vi "DiffDriveTrainSim_Update.vi"(6 "dT_Seconds":dbl=0.02, 11 "in DiffDriveTrainSim":T1 {"m_Motor"."Jr_KgM2" format="%13.5p"; "m_Motor"."L_H" format="%13.5p"; "m_Motor"."Kt_NMPerAmp" format="%13.5p"; "m_Motor"."KvINV_RadPerSecPerVolt" format="%13.5p"; "m_Motor"."R_Ohms" format="%13.5p"; "m_Motor"."FreeSpeed_RadPerSec" format="%13.5p"; "m_Motor"."FreeCurrent_Amps" format="%13.5p"; "m_Motor"."StallCurrent_Amps" format="%13.5p"; "m_Motor"."StallTorque_NM" format="%13.5p"; "m_Motor"."nominalVoltage_Volts" format="%13.5p"}) -> (0 "Error":bool, 3 "out DiffDriveTrainSim":T1 {"m_Motor"."Jr_KgM2" format="%13.5p"; "m_Motor"."L_H" format="%13.5p"; "m_Motor"."Kt_NMPerAmp" format="%13.5p"; "m_Motor"."KvINV_RadPerSecPerVolt" format="%13.5p"; "m_Motor"."R_Ohms" format="%13.5p"; "m_Motor"."FreeSpeed_RadPerSec" format="%13.5p"; "m_Motor"."FreeCurrent_Amps" format="%13.5p"; "m_Motor"."StallCurrent_Amps" format="%13.5p"; "m_Motor"."StallTorque_NM" format="%13.5p"; "m_Motor"."nominalVoltage_Volts" format="%13.5p"})   [LabVIEW 2019, in "Trajectory_Library.lvlib"]
doc: "Update the drivetrain states with the current time difference.\n \nInputs:\n - DiffDriveTraimSim -- Data cluster\n - dtSeconds -- the time difference\n\nOutputs:\n - OutDiffDriveTraimSim -- Updated data cluster.\n - Error -- If TRUE, an error occured."
uses:
  Trajectory_Library.lvlib
  TypeDef/DIFF_DRIVE_TRAIN_SIM.ctl
  TypeDef/LINEAR_SYSTEM.ctl
  <vilib>/Analysis/Matrix/Datatypes/RealMatrix.ctl
  TypeDef/DCMOTOR.CTL
  MatrixHelper_CoerceSize.vi
  MatBuilder_Create.vi
  <vilib>/Analysis/1siggen.llb/Gaussian White Noise.vi
  <vilib>/Analysis/Matrix/Numeric/Add/Add - RM,RM.vi
  <vilib>/Analysis/Matrix/NI_Matrix.lvlib
panel:
  # "<States, 1>"
  # "<Outputs, 1>"
  # "<Inputs, 1>"
  # "<Outputs, 1>"
  # "<States,States>"
  # "<States,Inputs>"
  # "<Outputs,States>"
  # "<Outputs,Inputs>"
  # "<States, 1>"
  # "<Outputs, 1>"
  # "<Inputs, 1>"
  # "<Outputs, 1>"
  # "<States,States>"
  # "<States,Inputs>"
  # "<Outputs,States>"
  # "<Outputs,Inputs>"
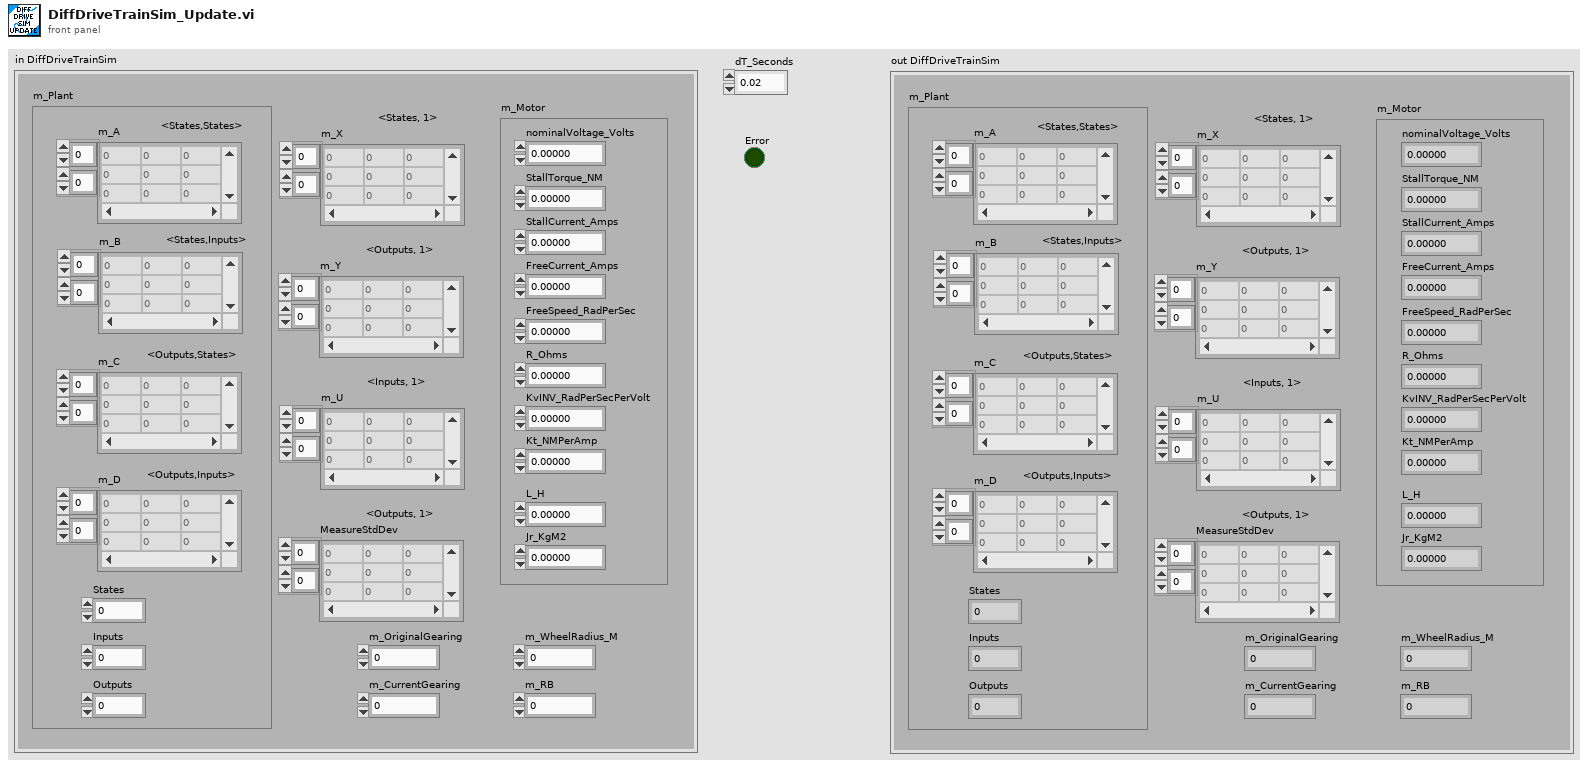
[diagram p1: front panel]
types:
  T1 = typedef "Trajectory_Library.lvlib/DIFF_DRIVE_TRAIN_SIM.ctl" = cluster{"m_Plant":T2, "m_X":T3, "m_Y":T3, "m_U":T3, "MeasureStdDev":T3, "m_Motor":T4, "m_OriginalGearing":dbl, "m_CurrentGearing":dbl, "m_WheelRadius_M":dbl, "m_RB":dbl}
  T2 = typedef "Trajectory_Library.lvlib/LINEAR_SYSTEM.ctl" = cluster{"m_A":T3, "m_B":T3, "m_C":T3, "m_D":T3, "States":i32, "Inputs":i32, "Outputs":i32}
  T3 = typedef "NI_Matrix.lvlib/RealMatrix.ctl" = dbl[][]
  T4 = typedef "Trajectory_Library.lvlib/DCMOTOR.CTL" = cluster{"nominalVoltage_Volts":dbl, "StallTorque_NM":dbl, "StallCurrent_Amps":dbl, "FreeCurrent_Amps":dbl, "FreeSpeed_RadPerSec":dbl, "R_Ohms":dbl, "KvINV_RadPerSecPerVolt":dbl, "Kt_NMPerAmp":dbl, "L_H":dbl, "Jr_KgM2":dbl}
  T5 = cluster{"m_A":T3, "m_B":T3, "m_CurrentGearing":dbl, "m_OriginalGearing":dbl, "m_RB":dbl}
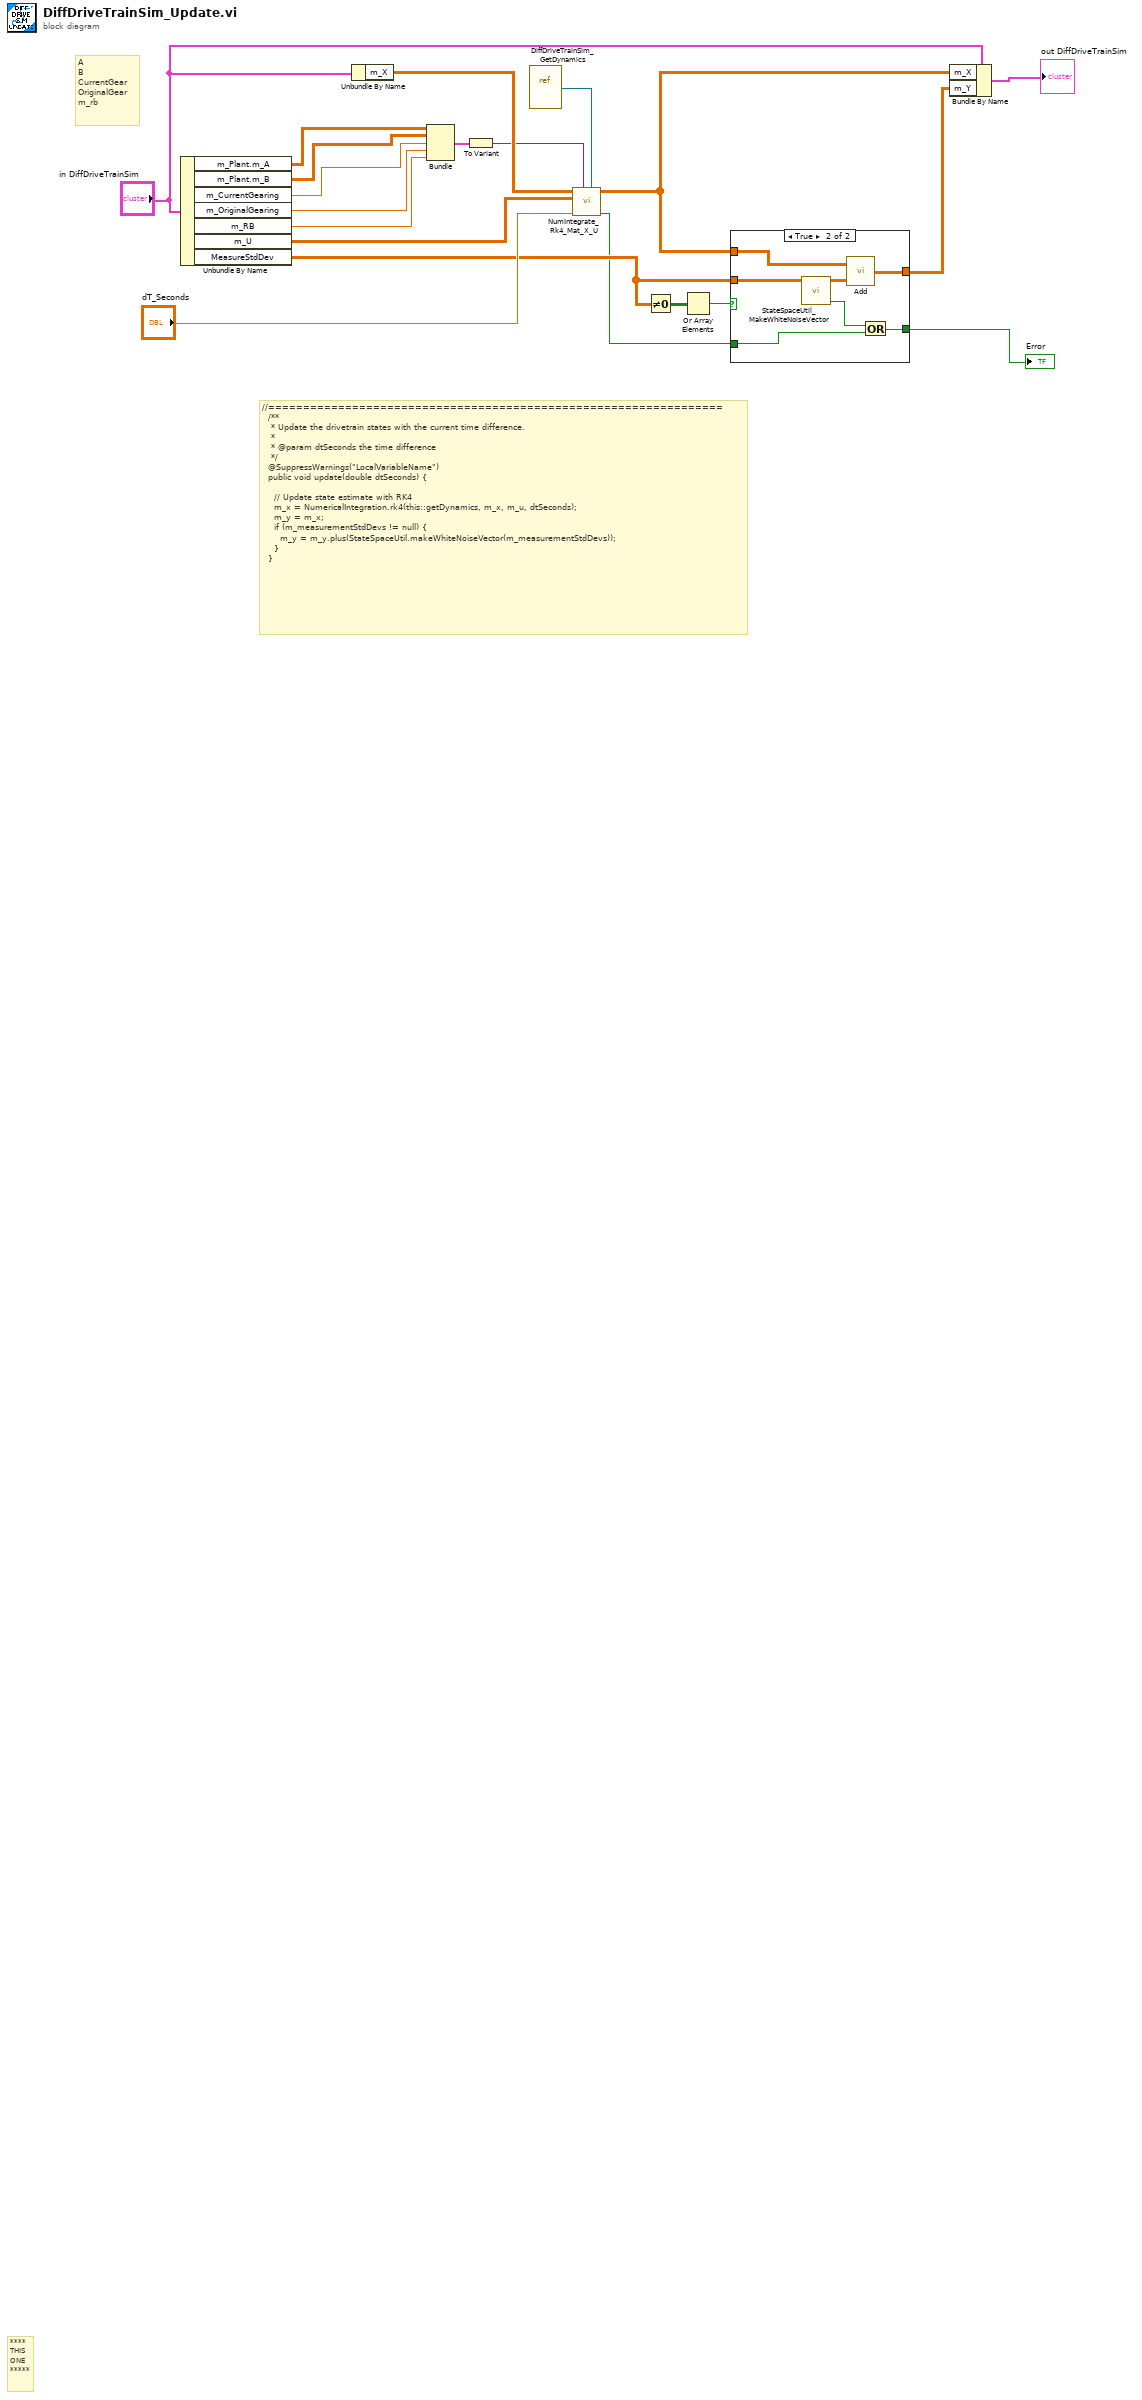
[diagram p0: block diagram]
diagram:
  # "A\nB\nCurrentGear\nOriginalGear\nm_rb"
  # "//=================================================================\n  /**\n   * Update the drivetrain states with the current time difference.\n   *\n   * @param dtSeconds the time difference\n   */\n  @SuppressWarnings(\"LocalVariableName\")\n  public void update(double dtSeconds) {\n\n    // Update state estimate with RK4\n    m_x = NumericalIntegration.rk4(this::getDynamics, m_x, m_u, dtSeconds);\n    m_y = m_x;\n    if (m_measurementStdDevs != null) {\n      m_y = m_y.plus(StateSpaceUtil.makeWhiteNoiseVector(m_measurementStdDevs));\n    }\n  }"
  # "****\nTHIS\nONE\n*****"
  n1 = Unbundle By Name("in DiffDriveTrainSim") -> ("m_Plant.m_A"=w15:T3, "m_Plant.m_B"=w14:T3, "m_CurrentGearing"=w13:dbl, "m_OriginalGearing"=w12:dbl, "m_RB"=w11:dbl, "m_U"=w20:T3, "MeasureStdDev"=w16:T3)
  n2 = Unbundle By Name("in DiffDriveTrainSim") -> ("m_X"=w5:T3)
  n3 = Bundle("m_A"=w15, "m_B"=w14, "m_CurrentGearing"=w13, "m_OriginalGearing"=w12, "m_RB"=w11) -> (w2:T5)  [unwired: 1 in]
  n4 = To Variant(anything=w2) -> (Variant=w3:variant)
  n5 = vi-ref "DiffDriveTrainSim_GetDynamics.vi"() -> (w4:refnum<vi>)
  n6 = call "NumIntegrate_Rk4_Mat_X_U.vi"("Func_X_U_Extra"=w4, "PassedData"=w3, "dT_Seconds"="dT_Seconds", "U"=w20, "X"=w5) -> ("Error"=w1:bool, "OUTPUT"=w6:T3)  [unwired: 5 in]
  n7 = Not Equal To 0?(x=w16) -> (x != 0?=w9:bool[][])
  n8 = Or Array Elements(Boolean array=w9) -> (logical OR=w8:bool)
  n9 = case shown="True" w8 {
    tunnel: w16 -> [_ w29]
    tunnel: w6 -> [w22 w27]
    tunnel: [w22 w26] -> w7
    tunnel: w1 -> [w21 w24]
    tunnel: [w21 w23] -> w10
    frame False {
    }
    frame True {
      n10 = call "StateSpaceUtil_MakeWhiteNoiseVector.vi"("StdDevs"=w29) -> ("Size Coerced"=w25:bool, "WhiteNoise"=w28:T3)  [unwired: 9 in]
      n11 = call-poly <vilib>:"Add.vi"("Real Matrix B"=w28, "Real Matrix A"=w27) -> ("A + B"=w26:T3)
      n12 = Or(x=w25, y=w24) -> (x .or. y?=w23:bool)
    }
  }
  "Error" <- w10
  n13 = Bundle By Name(cluster="in DiffDriveTrainSim", "m_X"=w6, "m_Y"=w7) -> (→"out DiffDriveTrainSim":T1)
